vi "_nicrio_cRIO-9217_UpdateConfigBox.vi"(8 "error in (no error)":errorcluster, 9 "_9217 Config":T1={"Conversion Time"=0, "Degree Range"=[], "RTD_Type"=[1], "RTD_A"=[], "RTD_B"=[], "RTD_C"=[], "RTD_Ro"=[]} {"RTD_Type" items=["TCR3851"=1, "TCR3750"=2, "TCR3916"=3, "TCR3920"=4, "TCR3911"=5, "TCR3928"=6, "Custom"=0]; "Degree Range" items=["Raw Ohms", "Degrees Kelvin", "Degrees Celsius", "Degrees Fahrenheit", "Degrees Rankine"]; "Conversion Time" items=["200 ms", "2.5 ms"]}, 11 "_Channel Refnum":refnum<vi>) -> (0 "error out":errorcluster)   [LabVIEW 2020, in "Modules.lvlib" / "9217.lvclass"]
uses:
  9217.lvclass
panel:
  in  "RTD Type":u8(ring) items=["TCR3851"=1, "TCR3750"=2, "TCR3916"=3, "TCR3920"=4, "TCR3911"=5, "TCR3928"=6, "Custom"=0]
  in  "Degree Range":u8(ring) items=["Raw Ohms", "Degrees Kelvin", "Degrees Celsius", "Degrees Fahrenheit", "Degrees Rankine"]
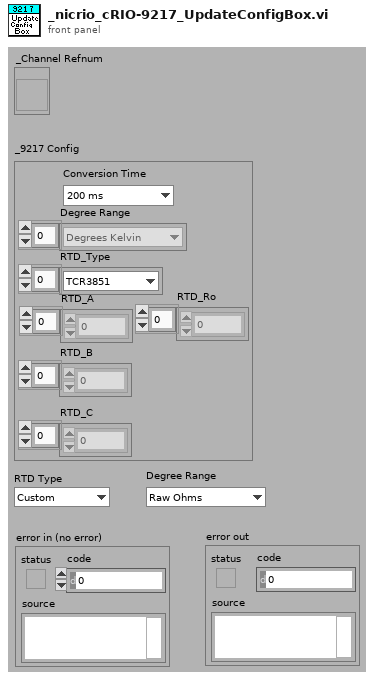
[diagram p1: front panel]
types:
  T1 = cluster{"Conversion Time":u16, "Degree Range":u8[], "RTD_Type":u8[], "RTD_A":dbl[], "RTD_B":dbl[], "RTD_C":dbl[], "RTD_Ro":dbl[]}
  T2 = typedef "LVStringsAndValuesArrayTypeDef_U8.ctl" = cluster{"String":string, "Value":u8}[]
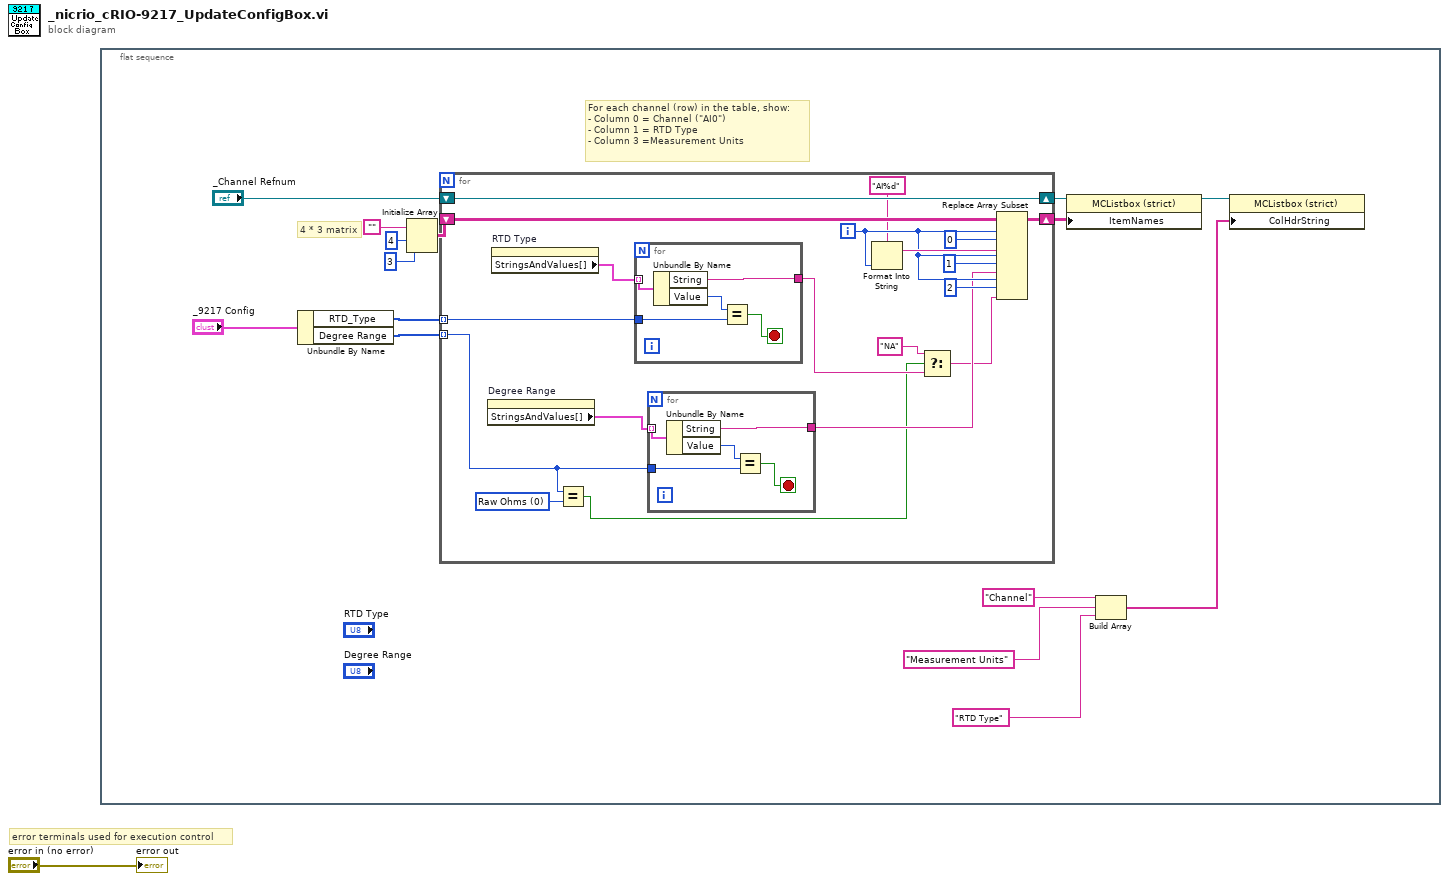
[diagram p0: block diagram]
diagram:
  # "error terminals used for execution control"
  n1 = flat-sequence {
    frame #0 {
      # "4 * 3 matrix"
      # "For each channel (row) in the table, show:\n- Column 0 = Channel (\"AI0\")\n- Column 1 = RTD Type\n- Column 3 =Measurement Units"
      n2 = Unbundle By Name("_9217 Config") -> ("RTD_Type"=w7:u8[], "Degree Range"=w6:u8[])
      n3 = Initialize Array("", 4 ("dimension size"), 3 ("dimension size")) -> (w13:string[][])
      n4 = for {
        shift-right: [w33] -> w16
        shift-left: w13 -> [w32]
        shift-right: [w35] -> w15
        shift-left: "_Channel Refnum" -> [w35]
        tunnel: w7 -> [w23] mode=indexing
        tunnel: w6 -> [w22] mode=indexing
        i -> [w28]
        w21 = u8 0 items=["Raw Ohms", "Degrees Kelvin", "Degrees Celsius", "Degrees Fahrenheit", "Degrees Rankine"] ("y")
        n5 = property on="Degree Range" class="Ring (strict)"() -> ("StringsAndValues[]"=w25:T2)  [unwired: 2 in, 2 out]
        n6 = property on="RTD Type" class="Ring (strict)"() -> ("StringsAndValues[]"=w26:T2)  [unwired: 2 in, 2 out]
        n7 = Equal?(x=w22, y=w21) -> (x = y?=w19:bool)
        n8 = for {
          tunnel: w26 -> [w45] mode=indexing
          tunnel: w23 -> [w43]
          tunnel: [w41] -> w20
          stop <- w42 stop-if-true
          n9 = Unbundle By Name(w45) -> ("String"=w41:string, "Value"=w44:u8)
          n10 = Equal?(x=w44, y=w43) -> (x = y?=w42:bool)
        }
        n11 = for {
          tunnel: w25 -> [w40] mode=indexing
          tunnel: w22 -> [w38]
          tunnel: [w36] -> w24
          stop <- w37 stop-if-true
          n12 = Unbundle By Name(w40) -> ("String"=w36:string, "Value"=w39:u8)
          n13 = Equal?(x=w39, y=w38) -> (x = y?=w37:bool)
        }
        n14 = Format Into String(format string="AI%d", w28) -> (resulting string=w29:string)  [unwired: 2 in, 1 out]
        n15 = Select(t="NA" ("Section"), s=w19, f=w20) -> (s? t:f=w18:string)
        n16 = Replace Array Subset(array=w32, new element #1=w29, index (row) #1=w28, index (col) #1=0 ("Column 1"), new element #2=w24, index (row) #2=w28, index (col) #2=1 ("Column 1"), new element #3=w18, index (row) #3=w28, index (col) #3=2 ("disabled index (col)")) -> (w33:string[][])
      }
      n17 = property on="Property Node" class="MCListbox (strict)"(reference=w15, "ItemNames"=w16) -> (reference out=w10:refnum<vi>)  [unwired: 1 in, 1 out]
      n18 = Build Array("Channel" ("Section"), "Measurement Units" ("String ID"), "RTD Type" ("String ID")) -> (w5:string[])
      n19 = property on="Property Node" class="MCListbox (strict)"(reference=w10, "ColHdrString"=w5) -> ()  [unwired: 1 in, 2 out]
    }
  }
  "error out" <- "error in (no error)"
